vi "Open Modbus.vi"(8 "error in (no error)":errorcluster, 11 "Modbus_Master in":refnum<class "Modbus_Master.lvclass">) -> (0 "error out":errorcluster, 3 "Modbus_Master out":refnum<class "Modbus_Master.lvclass">)   [LabVIEW 2021, in "Modbus_Master.lvclass"]
uses:
  Modbus_Master.lvclass
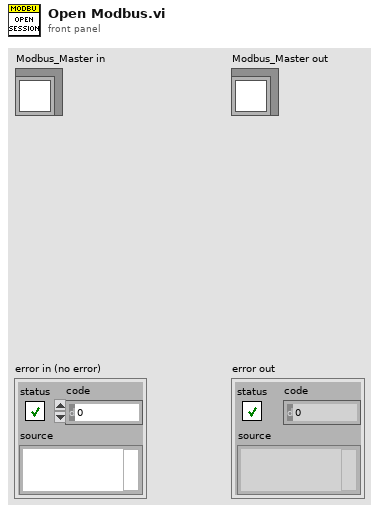
[diagram p1: front panel]
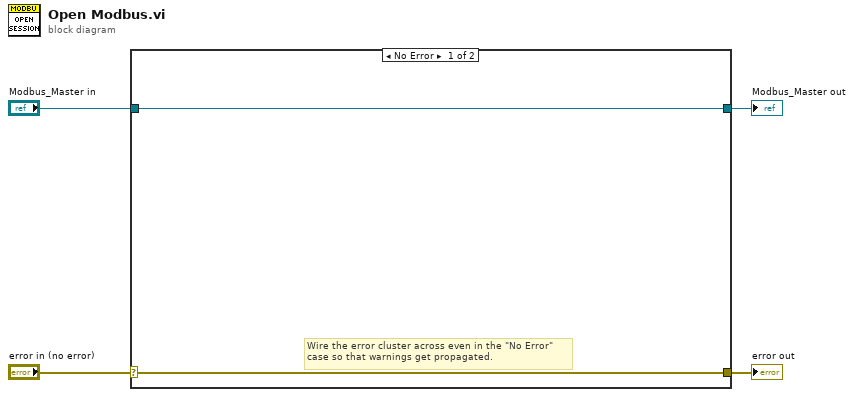
[diagram p0: block diagram]
diagram:
  n1 = case shown="No Error" "error in (no error)" {
    selector: "error in (no error)" -> [w5 w8]
    tunnel: [w5 w8] -> w3
    tunnel: [w6 w7] -> w1
    tunnel: "Modbus_Master in" -> [w6 w7]
    frame No Error {
      # "Wire the error cluster across even in the \"No Error\"\ncase so that warnings get propagated."
    }
    frame Error {
    }
  }
  "error out" <- w3
  "Modbus_Master out" <- w1
